vi "Write.vi"(8 "error in (no error)":errorcluster, 10 "data in":dbl, 11 "Modbus_AO in":refnum<class "Modbus_AO.lvclass">) -> (0 "error out":errorcluster, 3 "Modbus_AO out":refnum<class "Modbus_AO.lvclass">)   [LabVIEW 2021, in "Modbus_AO.lvclass"]
uses:
  Modbus_AO.lvclass
  Modbus_AO.lvclass/Modbus_AO.ctl
  Modbus_Master/Modbus_Master.lvclass
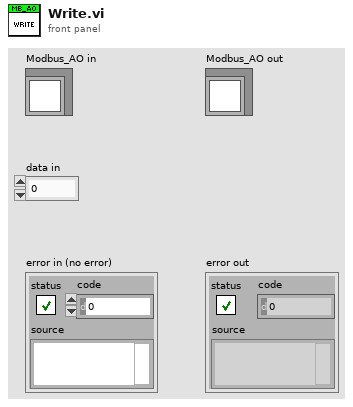
[diagram p1: front panel]
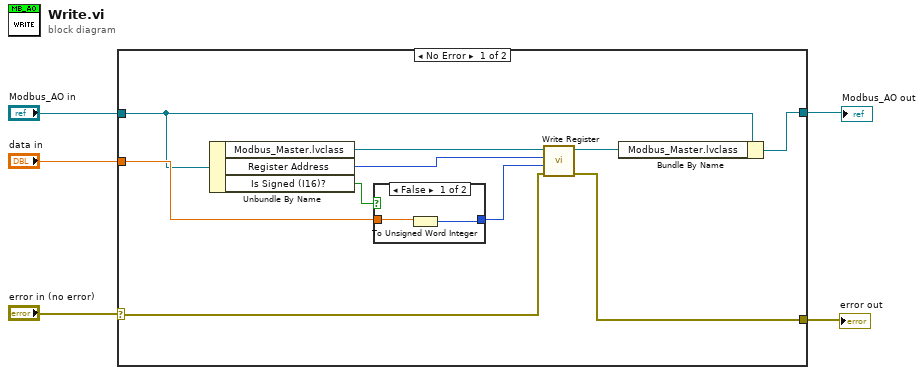
[diagram p0: block diagram]
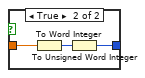
[diagram p2: hidden frame]
diagram:
  n1 = case shown="No Error" "error in (no error)" {
    selector: "error in (no error)" -> [w10 w21]
    tunnel: "Modbus_AO in" -> [w9 w22]
    tunnel: "data in" -> [w14 _]
    tunnel: [w7 w21] -> w2
    tunnel: [w6 w22] -> w1
    frame No Error {
      n2 = Unbundle By Name(w9) -> ("Modbus_Master.lvclass"=w12:refnum<class "Modbus_Master.lvclass">, "Register Address"=w11:u16, "Is Signed (I16)?"=w15:bool)
      n3 = case shown="False" w15 {
        tunnel: w14 -> [w17 w20]
        tunnel: [w16 w18] -> w13
        frame False {
          n4 = To Unsigned Word Integer(number=w17) -> (unsigned 16bit integer=w16:u16)
        }
        frame True {
          n5 = To Word Integer(number=w20) -> (16bit integer=w19:i16)
          n6 = To Unsigned Word Integer(number=w19) -> (unsigned 16bit integer=w18:u16)
        }
      }
      n7 = call "Write Register.vi"("error in (no error)"=w10, "Value"=w13, "Register Address"=w11, "Modbus_Master in"=w12) -> ("error out"=w7:errorcluster, "Modbus_Master out"=w8:refnum<class "Modbus_Master.lvclass">)  [unwired: 6 in]
      n8 = Bundle By Name(cluster=w9, "Modbus_Master.lvclass"=w8) -> (w6:refnum<class "Modbus_AO.lvclass">)
    }
    frame Error {
    }
  }
  "error out" <- w2
  "Modbus_AO out" <- w1
